vi "set Display Line.vi"(8 "error in (no error)":errorcluster, 9 "Line Index":i32, 10 "Amplitude":dbl, 11 "Keysight 9020A in":refnum<class "Keysight 9020A.lvclass">) -> (0 "error out":errorcluster, 3 "Keysight 9020A out":refnum<class "Keysight 9020A.lvclass">)   [LabVIEW 2023, in "Spectrum Analyzer.lvlib" / "Keysight 9020A.lvclass"]
uses:
  Keysight 9020A.lvclass
  Keysight 9020A.lvclass/Keysight 9020A.ctl
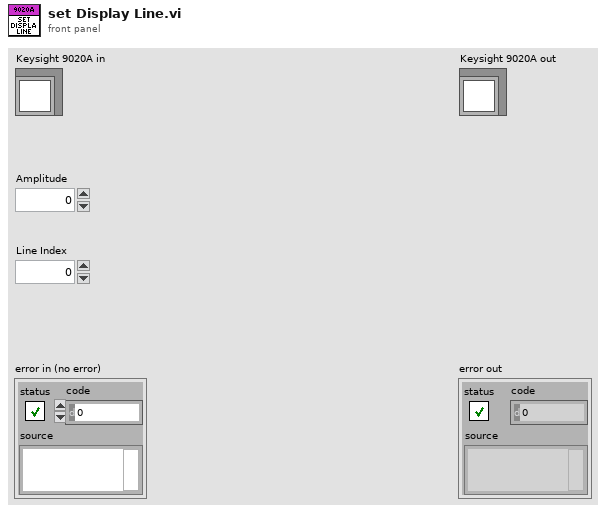
[diagram p1: front panel]
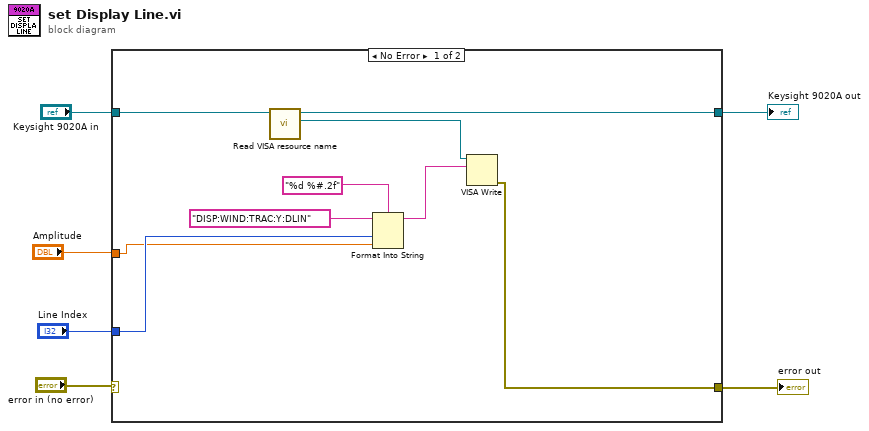
[diagram p0: block diagram]
diagram:
  n1 = case shown="No Error" "error in (no error)" {
    selector: "error in (no error)" -> [_ w16]
    tunnel: "Keysight 9020A in" -> [w11 w17]
    tunnel: [w15 w17] -> w5
    tunnel: [w7 w16] -> w1
    tunnel: "Amplitude" -> [w8 _]
    tunnel: "Line Index" -> [w9 _]
    frame No Error {
      n2 = call "Read VISA resource name.vi"("Keysight 9020A in"=w11) -> ("VISA resource name"=w12:refnum<visa-resource-name>, "Keysight 9020A out"=w15:refnum<class "Keysight 9020A.lvclass">)  [unwired: 8 in, 1 out]
      n3 = Format Into String(format string="%d %#.2f", initial string="DISP:WIND:TRAC:Y:DLIN", w9, w8) -> (resulting string=w14:string)  [unwired: 1 in, 1 out]
      n4 = VISA Write(VISA resource name=w12, write buffer=w14) -> (error out=w7:errorcluster)  [unwired: 1 in, 2 out]
    }
    frame Error {
    }
  }
  "error out" <- w1
  "Keysight 9020A out" <- w5
